vi "data to read.vi"(7 "Station":string(combo)="Load", 10 "Write data":u8[](array[numeric]), 11 "read data":u8[](array[numeric])) -> (1 "test state":T2, 2 "string":T1, 4 "result":bool[](array[boolean]))   [LabVIEW 2013]
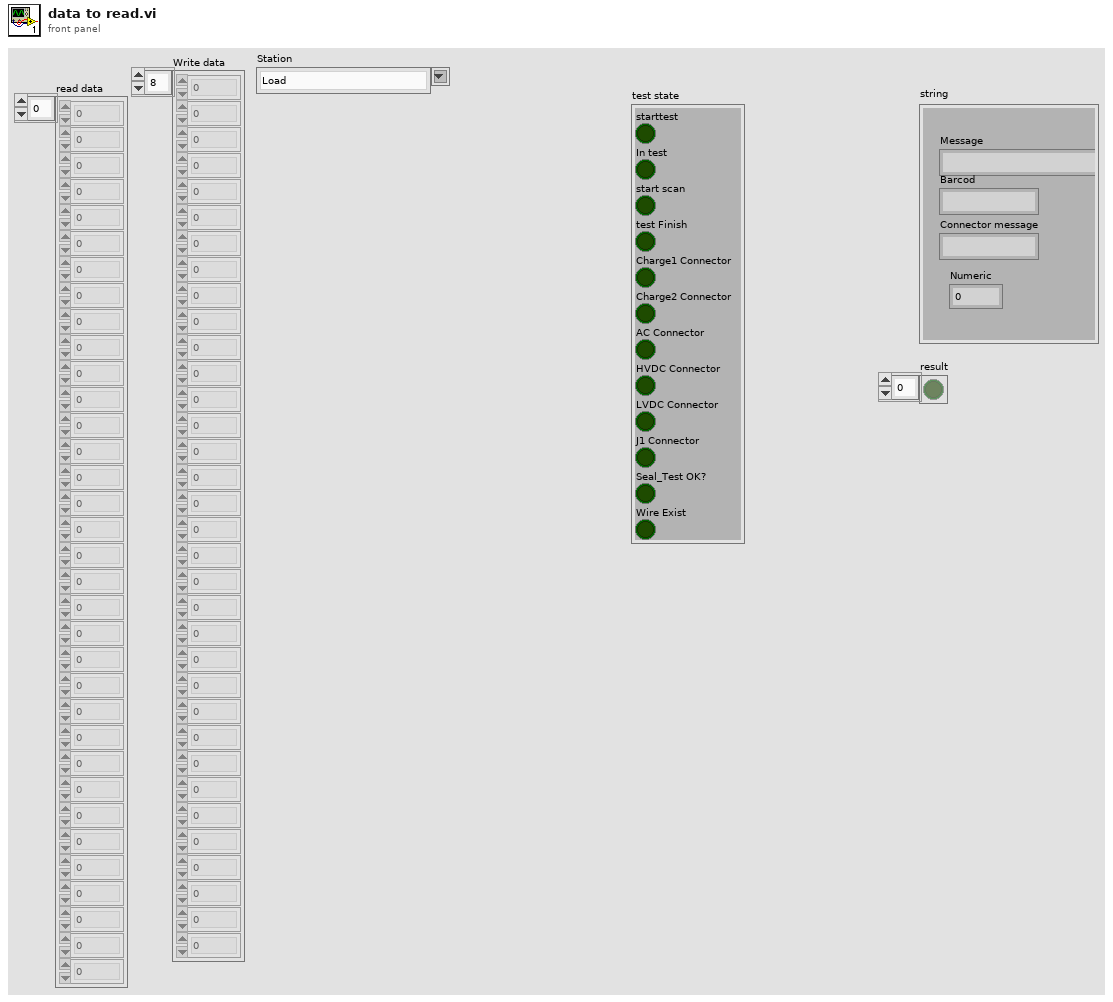
[diagram p1: front panel]
types:
  T1 = cluster{"Message":string, "Barcod":string, "Connector message":string, "Numeric":dbl}
  T2 = cluster{"starttest":bool, "In test":bool, "start scan":bool, "test Finish":bool, "Charge1 Connector":bool, "Charge2 Connector":bool, "AC Connector":bool, "HVDC Connector":bool, "LVDC Connector":bool, "J1 Connector":bool, "Seal_Test OK?":bool, "Wire Exist":bool}
  T3 = cluster{"format string":string, "type":enum16{"Error", "Alrm", "Warning", "Tips"}}[]
  T4 = cluster{"format string":string, "type":enum16{"Error", "Alrm", "Warning", "Tips"}}
  T5 = cluster{"[0]":bool, "[1]":bool, "[2]":bool, "[3]":bool, "[4]":bool, "[5]":bool, "[6]":bool, "[7]":bool, "[8]":bool, "[9]":bool, "[10]":bool, "[11]":bool}
  T6 = cluster{"string":string, "string":string, "substring":string, u16}
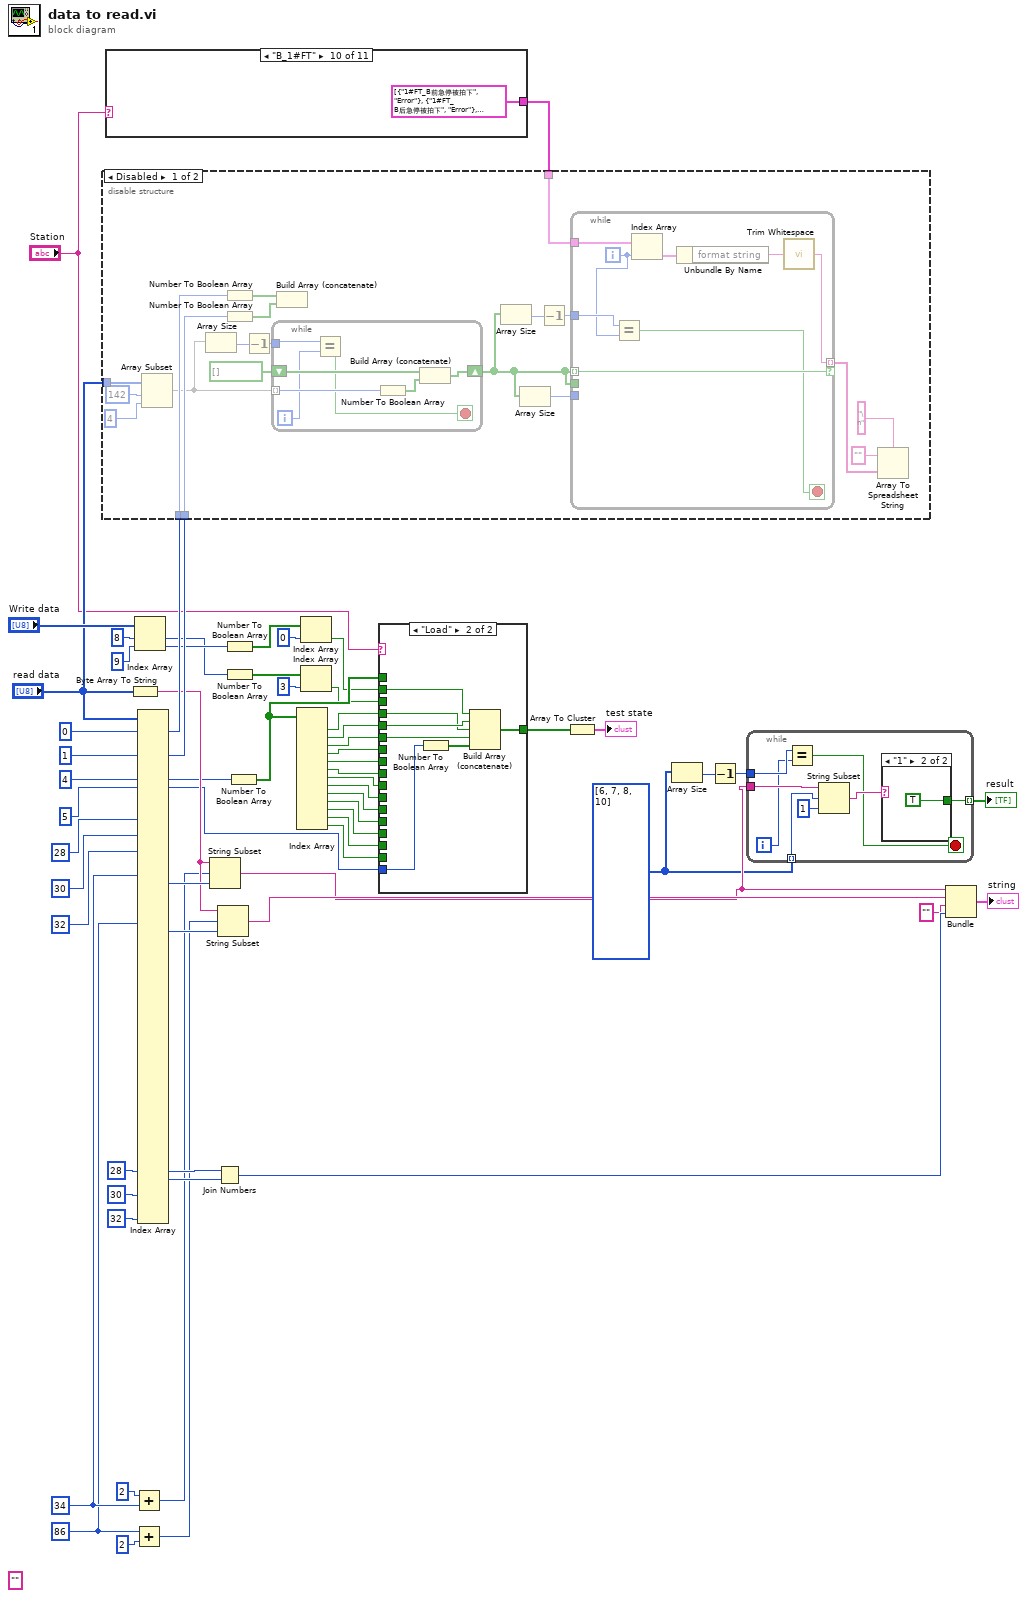
[diagram p0: block diagram]
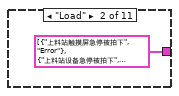
[diagram p5: hidden frame]
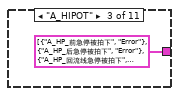
[diagram p6: hidden frame]
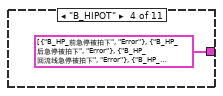
[diagram p7: hidden frame]
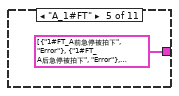
[diagram p8: hidden frame]
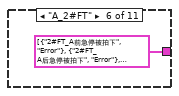
[diagram p9: hidden frame]
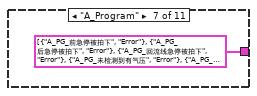
[diagram p10: hidden frame]
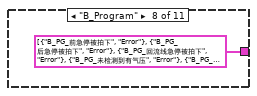
[diagram p11: hidden frame]
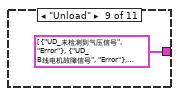
[diagram p12: hidden frame]
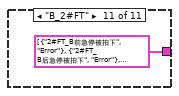
[diagram p13: hidden frame]
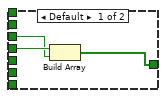
[diagram p14: hidden frame]
diagram:
  w2 = i32[] [6, 7, 8, 10]
  (unwired) "" ("format string")
  w55 = 34 ("index")
  w52 = 86 ("index")
  n1 = case shown="\"B_1#FT\"" "Station" {
    tunnel: [_ T3 [{"format string"="上料站触摸屏急停被拍下", "type"=enum."Error"}, {"format string"="上料站设备急停被拍下", "type"=enum."Error"}, {"format string"="前线右侧急停被拍下", "type"=enum."Error"}, {"format string"="后线左侧急停被拍下", "type"=enum."Error"}, {"format string"="后线右侧急停被拍下", "type"=enum."Error"}, {"format string"="未检测到气压信号", "type"=enum."Error"}, {"format string"="自动模式门锁打开", "type"=enum."Error"}, {"format string"="i_回流线电机故障信号", "type"=enum."Error"}, {"format string"="i_LD电机故障信号", "type"=enum."Error"}, {"format string"="i_前侧线电机故障信号", "type"=enum."Error"}, {"format string"="i_LD_A入料区电机故障信号", "type"=enum."Error"}, {"format string"="i_LD_B入料区电机故障信号", "type"=enum."Error"}, {"format string"="Charge1接头未到位报警", "type"=enum."Alrm"}, {"format string"="Charge2接头未到位报警", "type"=enum."Alrm"}, {"format string"="AC接头未到位报警", "type"=enum."Alrm"}, {"format string"="HVDC接头未到位报警", "type"=enum."Alrm"}, {"format string"="LVDC接头未到位报警", "type"=enum."Alrm"}, {"format string"="J1接头未到位报警", "type"=enum."Alrm"}, {"format string"="产品没有放平", "type"=enum."Alrm"}, {"format string"="RFID写入FAIL", "type"=enum."Alrm"}, {"format string"="扫码FAIL", "type"=enum."Alrm"}, {"format string"="上料站FIS_FAIL", "type"=enum."Alrm"}, {"format string"="RFID读取FAIL", "type"=enum."Alrm"}, {"format string"="门锁打开", "type"=enum."Warning"}, {"format string"="光栅遮挡", "type"=enum."Warning"}, {"format string"="PC未Ready", "type"=enum."Warning"}, {"format string"="泄露检测失败", "type"=enum."Warning"}, {"format string"="开关针气缸回原报警", "type"=enum."Alrm"}, {"format string"="开关针气缸进报警", "type"=enum."Alrm"}, {"format string"="开关针气缸既不在原位也不在工作位报警", "type"=enum."Alrm"}, {"format string"="上料站气路气缸回原报警", "type"=enum."Alrm"}, {"format string"="上料站气路气缸进报警", "type"=enum."Alrm"}, {"format string"="上料站气路气缸既不在原位也不在工作位报警", "type"=enum."Alrm"}, {"format string"="上料站顶升气缸回原报警", "type"=enum."Alrm"}, {"format string"="上料站顶升气缸进报警", "type"=enum."Alrm"}, {"format string"="上料站顶升气缸既不在原位也不在工作位报警", "type"=enum."Alrm"}, {"format string"="B线入料口顶升气缸回原报警", "type"=enum."Alrm"}, {"format string"="B线入料口顶升气缸进报警", "type"=enum."Alrm"}, {"format string"="B线入料口顶升气缸既不在原位也不在工作位报警", "type"=enum."Alrm"}, {"format string"="A线入料口顶升气缸进报警", "type"=enum."Alrm"}, {"format string"="A线入料口顶升气缸回原报警", "type"=enum."Alrm"}, {"format string"="A线入料口顶升气缸中位报警", "type"=enum."Alrm"}] ("Array 2") T3 [{"format string"="A_HP_前急停被拍下", "type"=enum."Error"}, {"format string"="A_HP_后急停被拍下", "type"=enum."Error"}, {"format string"="A_HP_回流线急停被拍下", "type"=enum."Error"}, {"format string"="A_HP_未检测到气压信号", "type"=enum."Error"}, {"format string"="A_HP_自动运行中前左门未关", "type"=enum."Error"}, {"format string"="A_HP_自动运行中前右门未关", "type"=enum."Error"}, {"format string"="A_HP_自动运行中后左门未关", "type"=enum."Error"}, {"format string"="A_HP_自动运行中后右门未关", "type"=enum."Error"}, {"format string"="A_HP_RFID读取FAIL", "type"=enum."Error"}, {"format string"="A_HP_RFID写入FAIL", "type"=enum."Error"}, {"format string"="A_HP_等待测试完成超时报警", "type"=enum."Error"}, {"format string"="A_HP_前侧左门开", "type"=enum."Error"}, {"format string"="A_HP_前侧右门开", "type"=enum."Error"}, {"format string"="A_HP_后侧左门开", "type"=enum."Error"}, {"format string"="A_HP_后侧右门开", "type"=enum."Error"}, {"format string"="A_HP_PC未Ready", "type"=enum."Error"}, {"format string"="A_HP_提升气缸回原报警", "type"=enum."Error"}, {"format string"="A_HP_提升气缸进报警", "type"=enum."Error"}, {"format string"="A_HP_提升气缸既不在工作位也不在原位", "type"=enum."Error"}, {"format string"="A_HP_辅助下降气缸回原报警", "type"=enum."Error"}, {"format string"="A_HP_辅助下降气缸进报警", "type"=enum."Error"}, {"format string"="A_HP_辅助下降气缸既不在工作位也不在原位", "type"=enum."Error"}, {"format string"="A_HP_辅助水平气缸回原报警", "type"=enum."Error"}, {"format string"="A_HP_辅助水平气缸进报警", "type"=enum."Error"}, {"format string"="A_HP_辅助水平气缸既不在工作位也不在原位", "type"=enum."Error"}, {"format string"="A_HP_AC测试气缸回原报警", "type"=enum."Error"}, {"format string"="A_HP_AC测试气缸进报警", "type"=enum."Error"}, {"format string"="A_HP_AC测试气缸既不在工作位也不在原位", "type"=enum."Error"}, {"format string"="A_HP_等待InTesting超时报警", "type"=enum."Error"}] ("Array 2") T3 [{"format string"="B_HP_前急停被拍下", "type"=enum."Error"}, {"format string"="B_HP_后急停被拍下", "type"=enum."Error"}, {"format string"="B_HP_回流线急停被拍下", "type"=enum."Error"}, {"format string"="B_HP_未检测到气压信号", "type"=enum."Error"}, {"format string"="B_HP_自动运行中前左门未关", "type"=enum."Error"}, {"format string"="B_HP_自动运行中前右门未关", "type"=enum."Error"}, {"format string"="B_HP_自动运行中后左门未关", "type"=enum."Error"}, {"format string"="B_HP_自动运行中后右门未关", "type"=enum."Error"}, {"format string"="B_HP_RFID读取FAIL", "type"=enum."Error"}, {"format string"="B_HP_RFID写入FAIL", "type"=enum."Error"}, {"format string"="B_HP_等待测试完成超时报警", "type"=enum."Error"}, {"format string"="B_HP_前侧左门开", "type"=enum."Error"}, {"format string"="B_HP_前侧右门开", "type"=enum."Error"}, {"format string"="BHP_后侧左门开", "type"=enum."Error"}, {"format string"="B_HP_后侧右门开", "type"=enum."Error"}, {"format string"="B_HP_PC未Ready", "type"=enum."Error"}, {"format string"="B_HP_提升气缸回原报警", "type"=enum."Error"}, {"format string"="B_HP_提升气缸进报警", "type"=enum."Error"}, {"format string"="B_HP_提升气缸既不在工作位也不在原位", "type"=enum."Error"}, {"format string"="B_HP_辅助下降气缸回原报警", "type"=enum."Error"}, {"format string"="B_HP_辅助下降气缸进报警", "type"=enum."Error"}, {"format string"="B_HP_辅助下降气缸既不在工作位也不在原位", "type"=enum."Error"}, {"format string"="B_HP_辅助水平气缸回原报警", "type"=enum."Error"}, {"format string"="B_HP_辅助水平气缸进报警", "type"=enum."Error"}, {"format string"="B_HP_辅助水平气缸既不在工作位也不在原位", "type"=enum."Error"}, {"format string"="B_HP_AC测试气缸回原报警", "type"=enum."Error"}, {"format string"="B_HP_AC测试气缸进报警", "type"=enum."Error"}, {"format string"="B_HP_AC测试气缸既不在工作位也不在原位", "type"=enum."Error"}, {"format string"="B_HP_等待InTesting超时报警", "type"=enum."Error"}] ("Array 2") T3 [{"format string"="1#FT_A前急停被拍下", "type"=enum."Error"}, {"format string"="1#FT_A后急停被拍下", "type"=enum."Error"}, {"format string"="1#FT_A回流线急停被拍下", "type"=enum."Error"}, {"format string"="1#FT_A未检测到有气压", "type"=enum."Error"}, {"format string"="1#FT_A自动运行过程中前左门被打开", "type"=enum."Error"}, {"format string"="1#FT_A自动运行过程中前右门被打开", "type"=enum."Error"}, {"format string"="1#FT_A自动运行过程中后左门被打开", "type"=enum."Error"}, {"format string"="1#FT_A自动运行过程中后右门被打开", "type"=enum."Error"}, {"format string"="1#FT_A自动流程中产生错误,请手动复位", "type"=enum."Error"}, {"format string"="RFID读取FAIL 110", "type"=enum."Alrm"}, {"format string"="RFID写入FAIL 120", "type"=enum."Alrm"}, {"format string"="等待测试完成超时报警 750", "type"=enum."Alrm"}, {"format string"="Q_HT_B前侧左门开", "type"=enum."Warning"}, {"format string"="Q_HT_B前侧右门开", "type"=enum."Warning"}, {"format string"="Q_HT_B后侧左门开", "type"=enum."Warning"}, {"format string"="Q_HT_B后侧右门开", "type"=enum."Warning"}, {"format string"="PC未Ready", "type"=enum."Warning"}, {"format string"="提升气缸回原报警", "type"=enum."Alrm"}, {"format string"="提升气缸进报警", "type"=enum."Alrm"}, {"format string"="提升气缸既不在工作位也不在原位报警", "type"=enum."Alrm"}, {"format string"="辅助升降气缸回原报警", "type"=enum."Alrm"}, {"format string"="辅助升降气缸进报警", "type"=enum."Alrm"}, {"format string"="辅助升降气缸既不在工作位也不在原位报警", "type"=enum."Alrm"}, {"format string"="辅助水平气缸回原报警", "type"=enum."Alrm"}, {"format string"="辅助水平气缸进报警", "type"=enum."Alrm"}, {"format string"="辅助水平气缸既不在工作位也不在原位报警", "type"=enum."Alrm"}, {"format string"="AC测试气缸回原报警", "type"=enum."Alrm"}, {"format string"="AC测试气缸进报警", "type"=enum."Alrm"}, {"format string"="AC测试气缸既不在工作位也不在原位报警", "type"=enum."Alrm"}, {"format string"="等待Intesting超时报警", "type"=enum."Error"}] ("Array 2") T3 [{"format string"="2#FT_A前急停被拍下", "type"=enum."Error"}, {"format string"="2#FT_A后急停被拍下", "type"=enum."Error"}, {"format string"="2#FT_A回流线急停被拍下", "type"=enum."Error"}, {"format string"="2#FT_A未检测到有气压", "type"=enum."Error"}, {"format string"="2#FT_A自动运行过程中前左门被打开", "type"=enum."Error"}, {"format string"="2#FT_A自动运行过程中前右门被打开", "type"=enum."Error"}, {"format string"="2#FT_A自动运行过程中后左门被打开", "type"=enum."Error"}, {"format string"="2#FT_A自动运行过程中后右门被打开", "type"=enum."Error"}, {"format string"="2#FT_A自动流程中产生错误,请手动复位 100", "type"=enum."Error"}, {"format string"="RFID读取报警 110", "type"=enum."Alrm"}, {"format string"="RFID写入报警 120", "type"=enum."Alrm"}, {"format string"="等待测试完成超时750", "type"=enum."Alrm"}, {"format string"="2#FT_A前侧左门开", "type"=enum."Warning"}, {"format string"="2#FT_A前侧右门开", "type"=enum."Warning"}, {"format string"="2#FT_A后侧左门开", "type"=enum."Warning"}, {"format string"="2#FT_A后侧右门开", "type"=enum."Warning"}, {"format string"="PC未Ready", "type"=enum."Warning"}, {"format string"="2#FT_A提升气缸回原报警", "type"=enum."Alrm"}, {"format string"="2#FT_A提升气缸进报警", "type"=enum."Alrm"}, {"format string"="2#FT_A提升气缸既不在原始位也不在工作位报警", "type"=enum."Alrm"}, {"format string"="2#FT_A辅助升降气缸回原报警", "type"=enum."Alrm"}, {"format string"="2#FT_A辅助升降气缸进报警", "type"=enum."Alrm"}, {"format string"="2#FT_A辅助升降气缸既不在原始位也不在工作位报警", "type"=enum."Alrm"}, {"format string"="2#FT_A辅助水平气缸回原报警", "type"=enum."Alrm"}, {"format string"="2#FT_A辅助水平气缸进报警", "type"=enum."Alrm"}, {"format string"="2#FT_A辅助水平气缸既不在原始位也不在工作位报警", "type"=enum."Alrm"}, {"format string"="2#FT_AAC测试气缸回原报警", "type"=enum."Alrm"}, {"format string"="2#FT_AAC测试气缸进报警", "type"=enum."Alrm"}, {"format string"="2#FT_AAC测试气缸既不在原始位也不在工作位报警", "type"=enum."Alrm"}, {"format string"="等待InTesting超时报警", "type"=enum."Error"}] ("Array 2") T3 [{"format string"="A_PG_前急停被拍下", "type"=enum."Error"}, {"format string"="A_PG_后急停被拍下", "type"=enum."Error"}, {"format string"="A_PG_回流线急停被拍下", "type"=enum."Error"}, {"format string"="A_PG_未检测到有气压", "type"=enum."Error"}, {"format string"="A_PG_自动运行过程中前左门被打开", "type"=enum."Error"}, {"format string"="A_PG_自动运行过程中前右门被打开", "type"=enum."Error"}, {"format string"="A_PG_自动运行过程中后左门被打开", "type"=enum."Error"}, {"format string"="A_PG_自动运行过程中后右门被打开", "type"=enum."Error"}, {"format string"="A_PG_自动流程中产生错误,请手动复位", "type"=enum."Error"}, {"format string"="RFID读取报警", "type"=enum."Alrm"}, {"format string"="RFID写入报警 120", "type"=enum."Alrm"}, {"format string"="测试等待超时 750", "type"=enum."Alrm"}, {"format string"="PG_A_前侧左门开", "type"=enum."Warning"}, {"format string"="PG_A_前侧右门开", "type"=enum."Warning"}, {"format string"="PG_A_后侧左门开", "type"=enum."Warning"}, {"format string"="PG_A_后侧右门开", "type"=enum."Warning"}, {"format string"="PC未Ready", "type"=enum."Warning"}, {"format string"="A_PG_提升气缸回原报警", "type"=enum."Alrm"}, {"format string"="A_PG_提升气缸进报警", "type"=enum."Alrm"}, {"format string"="A_PG_提升气缸既不在工作位也不在原位报警", "type"=enum."Alrm"}, {"format string"="等待InTesting超时报警", "type"=enum."Error"}] ("Array 2") T3 [{"format string"="B_PG_前急停被拍下", "type"=enum."Error"}, {"format string"="B_PG_后急停被拍下", "type"=enum."Error"}, {"format string"="B_PG_回流线急停被拍下", "type"=enum."Error"}, {"format string"="B_PG_未检测到有气压", "type"=enum."Error"}, {"format string"="B_PG_自动运行过程中前左门被打开", "type"=enum."Error"}, {"format string"="B_PG_自动运行过程中前右门被打开", "type"=enum."Error"}, {"format string"="B_PG_自动运行过程中后左门被打开", "type"=enum."Error"}, {"format string"="B_PG_自动运行过程中后右门被打开", "type"=enum."Error"}, {"format string"="B_PG_自动流程中产生错误,请手动复位", "type"=enum."Error"}, {"format string"="RFID读取报警", "type"=enum."Alrm"}, {"format string"="RFID写入报警 120", "type"=enum."Alrm"}, {"format string"="测试等待超时 750", "type"=enum."Alrm"}, {"format string"="PG_A_前侧左门开", "type"=enum."Warning"}, {"format string"="PG_A_前侧右门开", "type"=enum."Warning"}, {"format string"="PG_A_后侧左门开", "type"=enum."Warning"}, {"format string"="PG_A_后侧右门开", "type"=enum."Warning"}, {"format string"="PC未Ready", "type"=enum."Warning"}, {"format string"="B_PG_提升气缸回原报警", "type"=enum."Alrm"}, {"format string"="B_PG_提升气缸进报警", "type"=enum."Alrm"}, {"format string"="B_PG_提升气缸既不在工作位也不在原位报警", "type"=enum."Alrm"}, {"format string"="等待InTesting超时报警", "type"=enum."Error"}] ("Array 2") T3 [{"format string"="UD_未检测到气压信号", "type"=enum."Error"}, {"format string"="UD_B线电机故障信号", "type"=enum."Error"}, {"format string"="UD_B出口横移电机故障信号", "type"=enum."Error"}, {"format string"="UD_B检修门缓冲区电机故障信号", "type"=enum."Error"}, {"format string"="UD_B检修门电机故障信号", "type"=enum."Error"}, {"format string"="UD_A_A线电机故障信号", "type"=enum."Error"}, {"format string"="UD_A出口横移电机故障信号", "type"=enum."Error"}, {"format string"="UD_A贴标站电机故障信号", "type"=enum."Error"}, {"format string"="UD_A出口电机故障信号", "type"=enum."Error"}, {"format string"="RFID读取FAIL", "type"=enum."Error"}, {"format string"="PC未Ready", "type"=enum."Error"}, {"format string"="UD_B线出口顶升气缸回原报警", "type"=enum."Error"}, {"format string"="UD_B线出口顶升气缸进报警", "type"=enum."Error"}, {"format string"="UD_B线出口顶升气缸既不在工作位也不在原位报警", "type"=enum."Error"}, {"format string"="UD_检修门气缸进报警", "type"=enum."Error"}, {"format string"="UD_检修门气缸退报警", "type"=enum."Error"}, {"format string"="UD_检修门气缸既不在工作位也不在原位报警", "type"=enum."Error"}, {"format string"="UD_A线末端顶升气缸回原报警", "type"=enum."Error"}, {"format string"="UD_A线末端顶升气缸进报警", "type"=enum."Error"}, {"format string"="UD_A线末端顶升气缸既不在工作位也不在原位报警", "type"=enum."Error"}, {"format string"="UD_A贴标站顶升气缸回原报警", "type"=enum."Error"}, {"format string"="UD_A贴标站顶升气缸进报警", "type"=enum."Error"}, {"format string"="UD_A贴标站顶升气缸既不在工作位也不在原位报警", "type"=enum."Error"}] ("Array 2") T3 [{"format string"="1#FT_B前急停被拍下", "type"=enum."Error"}, {"format string"="1#FT_B后急停被拍下", "type"=enum."Error"}, {"format string"="1#FT_B未检测到有气压", "type"=enum."Error"}, {"format string"="1#FT_B自动运行过程中前左门被打开", "type"=enum."Error"}, {"format string"="1#FT_B自动运行过程中前右门被打开", "type"=enum."Error"}, {"format string"="1#FT_B自动运行过程中后左门被打开", "type"=enum."Error"}, {"format string"="1#FT_B自动运行过程中后右门被打开", "type"=enum."Error"}, {"format string"="1#FT_B自动流程中产生错误,请手动复位 100", "type"=enum."Error"}, {"format string"="1#FT_B_前阻挡RFID读取FAIL", "type"=enum."Alrm"}, {"format string"="1#FT_B_前阻挡RFID写入FAIL", "type"=enum."Alrm"}, {"format string"="1#FT_B前侧左门开", "type"=enum."Warning"}, {"format string"="1#FT_B前侧右门开", "type"=enum."Warning"}, {"format string"="1#FT_B后侧左门开", "type"=enum."Warning"}, {"format string"="1#FT_B后侧右门开", "type"=enum."Warning"}, {"format string"="1#FT_B_PC未Ready", "type"=enum."Warning"}, {"format string"="扫码FAIL", "type"=enum."Warning"}, {"format string"="1#FT_B小车锁紧气缸回原报警", "type"=enum."Alrm"}, {"format string"="1#FT_B小车锁紧气缸进报警", "type"=enum."Alrm"}, {"format string"="1#FT_B小车锁紧气缸既不在工作位也不在原位报警", "type"=enum."Alrm"}, {"format string"="1#FT_B提升气缸回原报警", "type"=enum."Alrm"}, {"format string"="1#FT_B提升气缸进报警", "type"=enum."Alrm"}, {"format string"="1#FT_B提升气缸既不在工作位也不在原位报警", "type"=enum."Alrm"}, {"format string"="1#FT_B辅助升降气缸回原报警", "type"=enum."Alrm"}, {"format string"="1#FT_B辅助升降气缸进报警", "type"=enum."Alrm"}, {"format string"="1#FT_B辅助升降气缸既不在工作位也不在原位报警", "type"=enum."Alrm"}, {"format string"="1#FT_B辅助水平气缸回原报警", "type"=enum."Alrm"}, {"format string"="1#FT_B辅助水平气缸进报警", "type"=enum."Alrm"}, {"format string"="1#FT_B辅助水平气缸既不在工作位也不在原位报警", "type"=enum."Alrm"}, {"format string"="1#FT_BAC测试气缸回原报警", "type"=enum."Alrm"}, {"format string"="1#FT_BAC测试气缸进报警", "type"=enum."Alrm"}, {"format string"="1#FT_BAC测试气缸既不在工作位也不在原位报警", "type"=enum."Alrm"}, {"format string"="1#FT_B_到位阻挡RFID读取FAIL", "type"=enum."Alrm"}, {"format string"="1#FT_B_到位阻挡RFID写入FAIL", "type"=enum."Alrm"}, {"format string"="等待InTesting超时报警", "type"=enum."Alrm"}, {"format string"="等待测试完成超时报警", "type"=enum."Alrm"}, {"format string"="", "type"=enum."Error"}] ("Array 2") T3 [{"format string"="2#FT_B前急停被拍下", "type"=enum."Error"}, {"format string"="2#FT_B后急停被拍下", "type"=enum."Error"}, {"format string"="2#FT_B未检测到有气压", "type"=enum."Error"}, {"format string"="2#FT_B自动运行过程中前左门被打开", "type"=enum."Error"}, {"format string"="2#FT_B自动运行过程中前右门被打开", "type"=enum."Error"}, {"format string"="2#FT_B自动运行过程中后左门被打开", "type"=enum."Error"}, {"format string"="2#FT_B自动运行过程中后右门被打开", "type"=enum."Error"}, {"format string"="2#FT_B自动流程中产生错误,请手动复位 ", "type"=enum."Error"}, {"format string"="2#FT_B_到位阻挡RFID读取FAIL 110", "type"=enum."Alrm"}, {"format string"="2#FT_B_到位阻挡RFID写入FAIL 120", "type"=enum."Alrm"}, {"format string"="2#FT_B前侧左门开", "type"=enum."Warning"}, {"format string"="2#FT_B前侧右门开", "type"=enum."Warning"}, {"format string"="2#FT_B后侧左门开", "type"=enum."Warning"}, {"format string"="2#FT_B后侧右门开", "type"=enum."Warning"}, {"format string"="PC未Ready", "type"=enum."Warning"}, {"format string"="2#FT_B后锁紧气缸回原报警", "type"=enum."Alrm"}, {"format string"="2#FT_B后锁紧气缸进报警", "type"=enum."Alrm"}, {"format string"="2#FT_B后锁紧气缸既不在工作位也不在原位报警", "type"=enum."Alrm"}, {"format string"="2#FT_B提升气缸回原报警", "type"=enum."Alrm"}, {"format string"="2#FT_B提升气缸进报警", "type"=enum."Alrm"}, {"format string"="2#FT_B提升气缸既不在工作位也不在原位报警", "type"=enum."Alrm"}, {"format string"="2#FT_B辅助升降气缸回原报警", "type"=enum."Alrm"}, {"format string"="2#FT_B辅助升降气缸进报警", "type"=enum."Alrm"}, {"format string"="2#FT_B辅助升降气缸既不在工作位也不在原位报警", "type"=enum."Alrm"}, {"format string"="2#FT_B辅助水平气缸回原报警", "type"=enum."Alrm"}, {"format string"="2#FT_B辅助水平气缸进报警", "type"=enum."Alrm"}, {"format string"="2#FT_B辅助水平气缸既不在工作位也不在原位报警", "type"=enum."Alrm"}, {"format string"="2#FT_BAC测试气缸回原报警", "type"=enum."Alrm"}, {"format string"="2#FT_BAC测试气缸进报警", "type"=enum."Alrm"}, {"format string"="2#FT_BAC测试气缸既不在工作位也不在原位报警", "type"=enum."Alrm"}, {"format string"="2#FT_B_后阻挡RFID读取FAIL 110", "type"=enum."Alrm"}, {"format string"="2#FT_B_后阻挡RFID写入FAIL 120", "type"=enum."Alrm"}, {"format string"="等待InTesting超时报警", "type"=enum."Alrm"}, {"format string"="等待测试完成超时报警", "type"=enum."Alrm"}] ("Array 2")] -> w7
    frame Default {
    }
    frame "Load" {
    }
    frame "A_HIPOT" {
    }
    frame "B_HIPOT" {
    }
    frame "A_1#FT" {
    }
    frame "A_2#FT" {
    }
    frame "A_Program" {
    }
    frame "B_Program" {
    }
    frame "Unload" {
    }
    frame "B_1#FT" {
    }
    frame "B_2#FT" {
    }
  }
  n2 = Byte Array To String(unsigned byte array="read data") -> (string=w53:string)
  n3 = Add(x=2, y=w55) -> (x+y=w21:i32)
  n4 = Add(x=w52, y=2) -> (x+y=w23:i32)
  n5 = Index Array(array="Write data", index #1=8 ("index"), index #2=9 ("index")) -> (element #1=w13:u8, element #2=w29:u8)
  n6 = Index Array(array="read data", index #1=0 ("index"), index #4=1 ("index"), index #7=4 ("index"), index #8=5 ("index"), index #12=28 ("index"), index #14=30 ("index"), index #16=32 ("index"), index #19=w55, index #25=w52, index #56=28 ("index"), index #59=30 ("index"), index #62=32 ("index")) -> (element #1=w63:u8, element #4=w61:u8, element #7=w16:u8, element #8=w15:u8, element #20=w54:u8, element #26=w51:u8, element #56=w25:u8, element #57=w24:u8)  [unwired: 50 in, 54 out]
  n7 = disable-structure shown="Disabled" {
    disable-tunnel: w63 -> [w93 _]
    disable-tunnel: w61 -> [w90 _]
    disable-tunnel: "read data" -> [w82 _]
    disable-tunnel: w7 -> [w81 _]
    frame Disabled {
      n8 = Array Subset(array=w82, index=142, length=4) -> (w79:u8[])
      n9 = Array Size(array=w79) -> (size(s)=w80:i32)
      n10 = Number To Boolean Array(number=w93) -> (Boolean array=w92:bool[])
      n11 = Number To Boolean Array(number=w90) -> (Boolean array=w91:bool[])
      n12 = Decrement(x=w80) -> (x-1=w78:i32)
      n13 = while {
        tunnel: w79 -> [w108] mode=indexing
        shift-right: [w105] -> w76
        shift-left: bool[] [] ("Boolean array") -> [w107]
        tunnel: w78 -> [w104]
        i -> [w103]
        stop <- w102 stop-if-true
        n14 = Equal?(x=w104, y=w103) -> (x = y?=w102:bool)
        n15 = Number To Boolean Array(number=w108) -> (Boolean array=w106:bool[])
        n16 = Build Array (concatenate)(w107, w106) -> (w105:bool[])
      }
      n17 = Build Array (concatenate)(w92, w91) -> ()  [unwired: 1 out]
      n18 = Array Size(array=w76) -> (size(s)=w77:i32)
      n19 = Array Size(array=w76) -> (size(s)=w83:i32)
      n20 = Decrement(x=w77) -> (x-1=w75:i32)
      n21 = while {
        tunnel: w76 -> [w101] mode=indexing
        tunnel: w81 -> [w98]
        tunnel: w76 -> [_]
        tunnel: [w99] -> w86 mode=indexing if=w101
        tunnel: w83 -> [_]
        tunnel: w75 -> [w96]
        i -> [w95]
        stop <- w94 stop-if-true
        n22 = Equal?(x=w96, y=w95) -> (x = y?=w94:bool)
        n23 = Index Array(array=w98, index=w95) -> (element=w97:T4)
        n24 = Unbundle By Name(w97) -> ("format string"=w100:string)
        n25 = call <vilib>:"Trim Whitespace.vi"("string"=w100) -> ("trimmed string"=w99:string)  [unwired: 1 in]
      }
      n26 = Array To Spreadsheet String(delimiter (Tab)="\n", array=w86, 3:"" ("format string")) -> ()  [unwired: 1 out]
    }
    frame Enabled {
    }
  }
  n27 = String Subset(string=w53, offset (0)=w21, length (rest)=w54) -> (substring=w5:string)
  n28 = Join Numbers(hi=w25, lo=w24) -> ((hi.lo)=w19:u16)
  n29 = String Subset(string=w53, offset (0)=w23, length (rest)=w51) -> (substring=w47:string)
  n30 = Number To Boolean Array(number=w29) -> (Boolean array=w28:bool[])
  n31 = Number To Boolean Array(number=w13) -> (Boolean array=w11:bool[])
  n32 = Number To Boolean Array(number=w16) -> (Boolean array=w30:bool[])
  n33 = Index Array(array=w30) -> (element #1=w46:bool, element #2=w45:bool, element #3=w41:bool, element #4=w40:bool, element #5=w39:bool, element #6=w38:bool, element #7=w37:bool, element #8=w36:bool, element #9=w35:bool, element #10=w34:bool, element #11=w33:bool, element #12=w32:bool, element #13=w31:bool)  [unwired: 13 in]
  n34 = Index Array(array=w28, index=0) -> (element=w26:bool)
  n35 = Index Array(array=w11, index=3) -> (element=w10:bool)
  n36 = case shown="\"Load\"" "Station" {
    tunnel: w46 -> [w111 w115]
    tunnel: w45 -> [_ w116]
    tunnel: [w110 w118] -> w44
    tunnel: w41 -> [_ w117]
    tunnel: w40 -> [_ _]
    tunnel: w39 -> [_ _]
    tunnel: w38 -> [_ _]
    tunnel: w37 -> [_ _]
    tunnel: w36 -> [_ _]
    tunnel: w35 -> [_ _]
    tunnel: w34 -> [_ _]
    tunnel: w33 -> [_ _]
    tunnel: w32 -> [_ _]
    tunnel: w31 -> [_ _]
    tunnel: w30 -> [_ _]
    tunnel: w26 -> [_ w112]
    tunnel: w15 -> [_ w114]
    tunnel: w10 -> [w109 _]
    frame Default {
      n37 = Build Array(w111, w109) -> (w110:bool[])
    }
    frame "Load" {
      n38 = Number To Boolean Array(number=w114) -> (Boolean array=w113:bool[])
      n39 = Build Array (concatenate)(w112, w116, w115, w117, w113) -> (w118:bool[])
    }
  }
  n40 = Array To Cluster(array=w44) -> (cluster=→"test state":T5)
  n41 = Array Size(array=w2) -> (size(s)=w3:i32)
  n42 = Decrement(x=w3) -> (x-1=w1:i32)
  n43 = while {
    tunnel: w5 -> [w126]
    tunnel: w2 -> [w124] mode=indexing
    tunnel: [w122] -> w4 mode=indexing
    tunnel: w1 -> [w121]
    i -> [w120]
    stop <- w119 stop-if-true
    n44 = Equal?(x=w121, y=w120) -> (x = y?=w119:bool)
    n45 = String Subset(string=w126, offset (0)=w124, length (rest)=1 ("length (rest)")) -> (substring=w123:string)
    n46 = case shown="\"1\"" w123 {
      tunnel: [_ TRUE] -> w122
      frame "False", Default {
      }
      frame "1" {
      }
    }
  }
  "result" <- w4
  n47 = Bundle("string"=w5, "string"=w47, "substring"="", w19) -> (→"string":T6)  [unwired: 1 in]
